vi "AutoMapClass.vi"(6 "Ignore if Not Found?":bool, 7 "SubPnl Refnum":refnum<vi>, 8 "error in (no error)":errorcluster, 9 "Payload":string, 10 "Command":string, 11 "Core Class":refnum<class>) -> (0 "error out":errorcluster, 2 "Response":string, 3 "Match Present?":bool)   [LabVIEW 2019, in "MicronServer.lvlib" / "Mapper.lvclass"]
uses:
  Mapper.lvclass
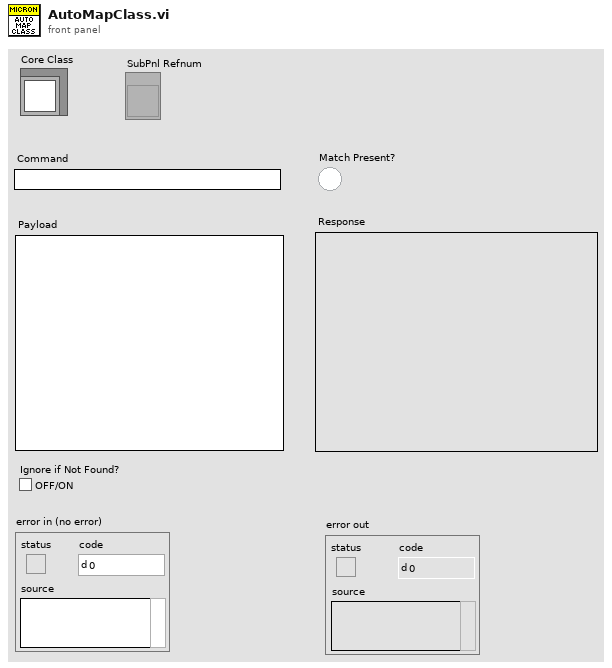
[diagram p1: front panel]
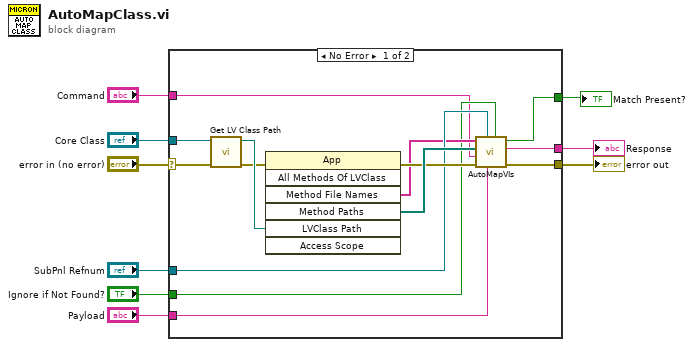
[diagram p0: block diagram]
diagram:
  n1 = case shown="No Error" "error in (no error)" {
    selector: "error in (no error)" -> [w17 w24]
    tunnel: "Core Class" -> [w23 _]
    tunnel: "Command" -> [w10 _]
    tunnel: "Payload" -> [w11 _]
    tunnel: [w20 _] -> w6
    tunnel: "SubPnl Refnum" -> [w14 _]
    tunnel: [w16 w24] -> w3
    tunnel: [w15 _] -> w2
    tunnel: "Ignore if Not Found?" -> [w12 _]
    frame No Error {
      n2 = call <vilib>:"Get LV Class Path.vi"("error in (no error)"=w17, "object"=w23) -> ("error out"=w19:errorcluster, "class path"=w22:path)  [unwired: 8 in]
      n3 = invoke class="App" method="All Methods Of LVClass"(error in=w19, "LVClass Path"=w22) -> (error out=w18:errorcluster, "Method File Names"=w13:string[], "Method Paths"=w21:path[])  [unwired: 5 in, 4 out]
      n4 = call "AutoMapVIs.vi"("Ignore if Not Found?"=w12, "Payload"=w11, "SubPanel in"=w14, "error in (no error)"=w18, "Command"=w10, "VI Paths"=w21, "Fully Qualified VI Names"=w13) -> ("error out"=w16:errorcluster, "Response"=w20:string, "Match Present?"=w15:bool)  [unwired: 2 in]
    }
    frame Error {
    }
  }
  "Response" <- w6
  "error out" <- w3
  "Match Present?" <- w2
